vi "Is Instrument a DCPower.vi"(9 "Instrument Name":string, 11 ".pinmap File Path":path) -> (3 "DCPower?":bool)   [LabVIEW 2025, in "Digital Pattern Sequencer.lvclass"]
uses:
  Digital Pattern Sequencer.lvclass
  Digital Pattern Sequencer.lvclass/Digital Pattern Sequencer.ctl
panel:
  out "offset of match":i32
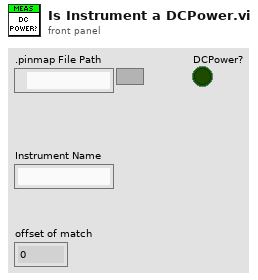
[diagram p1: front panel]
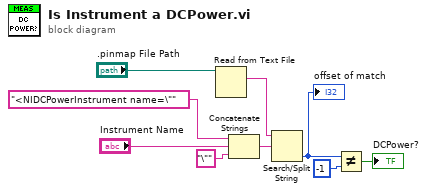
[diagram p0: block diagram]
diagram:
  n1 = Read from Text File(file (use dialog)=".pinmap File Path") -> (text=w5:string)  [unwired: 3 in, 3 out]
  n2 = Concatenate Strings("<NIDCPowerInstrument name=\"" ("string"), "Instrument Name", "\"" ("string")) -> (w4:string)
  n3 = Search/Split String(string=w5, search string/char (-)=w4) -> (offset of match=w3:i32)  [unwired: 1 in, 2 out]
  "offset of match" <- w3
  n4 = Not Equal?(x=w3, y=-1) -> (x != y?=→"DCPower?":bool)
